vi "Get Translations status symbol.vi"(9 "Property":T1[](array[typedef]), 10 "Not found":bool, 11 "Number Of Languages":i32) -> (0 "Item Symbol":i32, 4 "State":string)   [LabVIEW 2019, in "Language Editor.lvlib"]
doc: "- - -\nCopyright (c) 2026, Merecs Engineering GmbH"
uses:
  Language Editor.lvlib
  Language Selection/TypeDefs/Cluster PropertyTranslation.ctl
  Language Selection/TypeDefs/Enum Property Type.ctl
  Language Selection/Language Selection.lvlib
panel:
  # "Connector Pane"
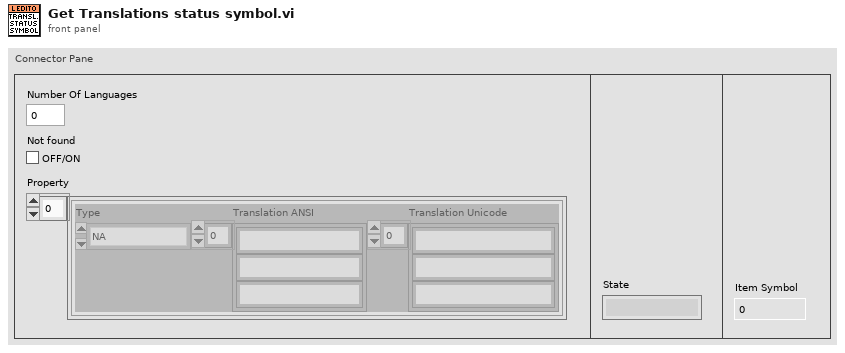
[diagram p1: front panel]
types:
  T1 = typedef "Language Selection.lvlib/Cluster PropertyTranslation.ctl" = cluster{"Type":T2, "Translation ANSI":string[], "Translation Unicode":string[]}
  T2 = typedef "Language Selection.lvlib/Enum Property Type.ctl" = enum16{"NA", "Caption", "String Value", "Boolean Text", "Ring Strings", "1D Array Elements", "2D Array Elements", "(MC)Listbox Header", "(MC)Listbox Items", "Tab Pages Names", "X & Y GraphChart", "Plot Names", "Table Headers", "Table Items", "TipStrip", "Combobox Strings", "Cursor Name", "Tree Col Headers"}
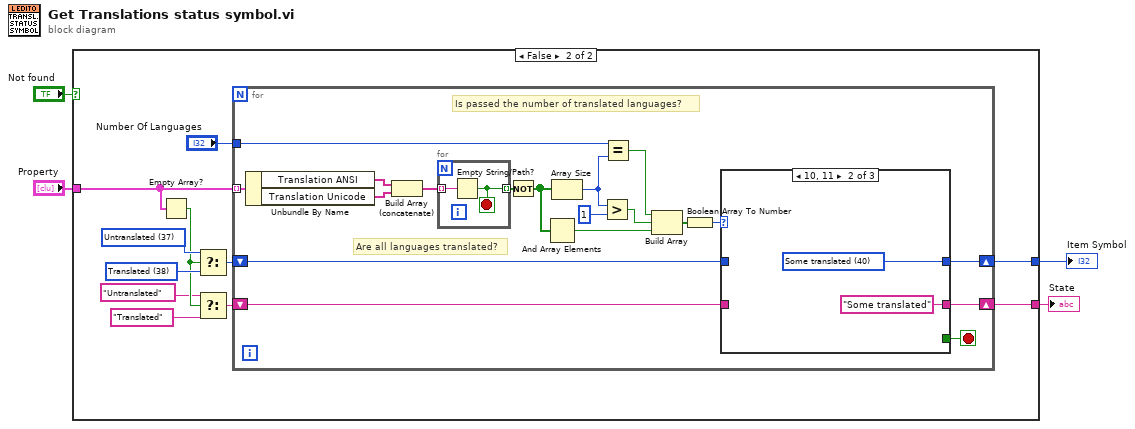
[diagram p0: block diagram]
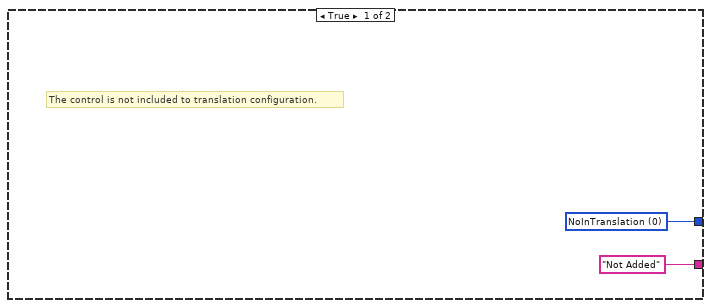
[diagram p2: hidden frame]
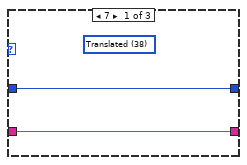
[diagram p3: hidden frame]
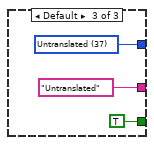
[diagram p4: hidden frame]
diagram:
  n1 = case shown="False" "Not found" {
    tunnel: [w6 w16] -> w4
    tunnel: "Property" -> [_ w15]
    tunnel: ["Not Added" w12] -> w3
    frame True {
      w6 = u16 0 items=["NoInTranslation"=0, "Untranslated"=37, "Translated"=38, "Some translated"=40]
      # "The control is not included to translation configuration."
    }
    frame False {
      w13 = u16 37 items=["NoInTranslation"=2, "Untranslated"=37, "Translated"=38, "Some translated"=40]
      w14 = u16 38 items=["Untranslated"=37, "Translated"=38, "Some translated"=40]
      n2 = Empty Array?(array=w15) -> (empty?=w10:bool)
      n3 = Select(t=w13, s=w10, f=w14) -> (s? t:f=w11:u16)
      n4 = Select(t="Untranslated", s=w10, f="Translated") -> (s? t:f=w9:string)
      n5 = for {
        tunnel: w15 -> [w36] mode=indexing
        tunnel: "Number Of Languages" -> [w33]
        shift-right: [w23] -> w16
        shift-left: w11 -> [w22]
        shift-right: [w19] -> w12
        shift-left: w9 -> [w18]
        stop <- w21 stop-if-true
        # "Are all languages translated?"
        # "Is passed the number of translated languages?"
        n6 = Unbundle By Name(w36) -> ("Translation ANSI"=w34:string[], "Translation Unicode"=w35:string[])
        n7 = Build Array (concatenate)(w34, w35) -> (w32:string[])
        n8 = for {
          tunnel: w32 -> [w45] mode=indexing
          tunnel: [w44] -> w27 mode=indexing
          stop <- w44 stop-if-true
          n9 = Empty String/Path?(string/path=w45) -> (empty?=w44:bool)
        }
        n10 = Not(x=w27) -> (.not. x?=w20:bool[])
        n11 = And Array Elements(Boolean array=w20) -> (logical AND=w28:bool)
        n12 = Array Size(array=w20) -> (size(s)=w25:i32)
        n13 = Greater?(x=w25, y=1) -> (0:w26:bool)
        n14 = Equal?(x=w33, y=w25) -> (x = y?=w31:bool)
        n15 = Build Array(w31, w26, w28) -> (w30:bool[])
        n16 = Boolean Array To Number(Boolean array=w30) -> (number=w29:u32)
        n17 = case shown="10, 11" w29 {
          tunnel: [w38 w40 w43] -> w23
          tunnel: w22 -> [w38 _ _]
          tunnel: [_ _ TRUE] -> w21
          tunnel: [w37 "Some translated" "Untranslated"] -> w19
          tunnel: w18 -> [w37 _ _]
          frame 7 {
            (unwired) u16 38 items=["Untranslated"=37, "Translated"=38, "Some translated"=40]
          }
          frame 2, 3 {
            w40 = u16 40 items=["Untranslated"=37, "Translated"=38, "Some translated"=40]
          }
          frame Default {
            w43 = u16 37 items=["Untranslated"=37, "Translated"=38, "Some translated"=40]
          }
        }
      }
    }
  }
  "Item Symbol" <- w4
  "State" <- w3
